vi "Finish Sequence.vi"(8 "error in":errorcluster, 11 "Sequence Executor in":refnum<class "Sequence Executor.lvclass">) -> (0 "error out":errorcluster, 3 "Sequence Executor out":refnum<class "Sequence Executor.lvclass">)   [LabVIEW 2026, in "Sequence Executor.lvclass"]
doc: "PRIVATE. Running F; verdict PASS iff every Step Result equals its step's expected_result; writes the CSV; applies safe setpoints to the rig; Status COMPLETE: verdict - file; refreshes displays."
uses:
  Sequence Executor.lvclass
  Sequence Executor.lvclass/Sequence Executor.ctl
  Rig Messages/Apply Setpoints Msg/Apply Setpoints Msg.lvclass/Apply Setpoints Msg.ctl
  <vilib>/ActorFramework/Message Enqueuer/Message Enqueuer.lvclass/Message Enqueuer.ctl
  <vilib>/ActorFramework/Message Enqueuer/Enqueue.vi
  Rig Messages/Apply Setpoints Msg/Apply Setpoints Msg.lvclass
  <vilib>/ActorFramework/Message Priority Queue/Priority Enqueue.vi
  <vilib>/ActorFramework/Message Enqueuer/Message Enqueuer.lvclass
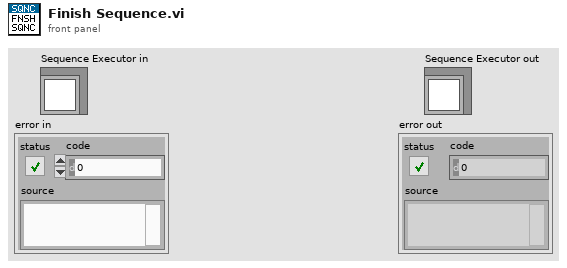
[diagram p1: front panel]
types:
  T1 = typedef "Step Result.ctl" = cluster{"step_no":i32, "step_name":string, "result":string, "reason":string, "measured":dbl, "target":dbl, "duration_ms":dbl}
  T2 = typedef "Sequence File.ctl" = cluster{"sequence_id":string, "description":string, "rig_config":string, "steps":T3[]}
  T3 = typedef "Step Config.ctl" = cluster{"step_no":i32, "step_name":string, "command_type":string, "setpoints":T4[], "conditions":T5[], "dwell_time_ms":i32, "timeout_ms":i32, "expected_result":string}
  T4 = typedef "Channel Value.ctl" = cluster{"channel":string, "value":dbl}
  T5 = typedef "Condition.ctl" = cluster{"channel":string, "target":dbl, "tolerance":dbl}
  T6 = typedef "Rig Config.ctl" = cluster{"rig_id":string, "description":string, "plugin_class":string, "channels":T7[]}
  T7 = typedef "Channel Definition.ctl" = cluster{"name":string, "unit":string, "min":dbl, "max":dbl}
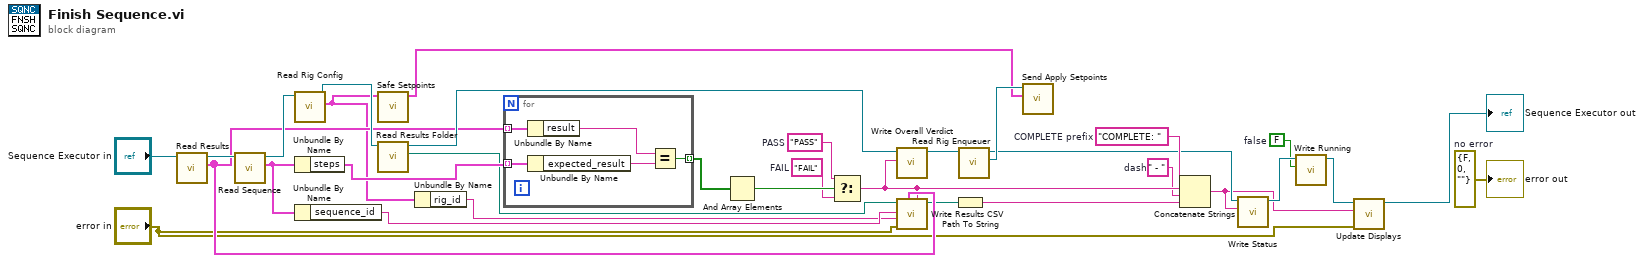
[diagram p0: block diagram]
diagram:
  w1 = FALSE  # false
  w10 = " - "  # dash
  w12 = "COMPLETE: "  # COMPLETE prefix
  w24 = "FAIL"  # FAIL
  w26 = "PASS"  # PASS
  w2 = errorcluster {"status"=FALSE, "code"=0, "source"=""}  # no error
  n1 = call "Read Results.vi"("Sequence Executor in"="Sequence Executor in") -> ("Results"=w18:T1[], "Sequence Executor out"=w31:refnum<class "Sequence Executor.lvclass">)  [unwired: 8 in, 1 out]
  n2 = call "Read Sequence.vi"("Sequence Executor in"=w31) -> ("Sequence File"=w22:T2, "Sequence Executor out"=w30:refnum<class "Sequence Executor.lvclass">)  [unwired: 8 in, 1 out]
  n3 = call "Read Rig Config.vi"("Sequence Executor in"=w30) -> ("Rig Config"=w17:T6, "Sequence Executor out"=w29:refnum<class "Sequence Executor.lvclass">)  [unwired: 8 in, 1 out]
  n4 = Unbundle By Name(w22) -> ("steps"=w28:T3[])
  n5 = Unbundle By Name(w22) -> ("sequence_id"=w20:string)
  n6 = call "Safe Setpoints.vi"("Rig Config"=w17) -> ("setpoints"=w14:cluster{"channel":string, "value":dbl}[])  [unwired: 10 in]
  n7 = call "Read Results Folder.vi"("Sequence Executor in"=w29) -> ("Results Folder"=w21:path, "Sequence Executor out"=w23:refnum<class "Sequence Executor.lvclass">)  [unwired: 8 in, 1 out]
  n8 = Unbundle By Name(w17) -> ("rig_id"=w19:string)
  n9 = for {
    tunnel: w18 -> [w37] mode=indexing
    tunnel: w28 -> [w36] mode=indexing
    tunnel: [w33] -> w27 mode=indexing
    n10 = Unbundle By Name(w37) -> ("result"=w35:string)
    n11 = Unbundle By Name(w36) -> ("expected_result"=w34:string)
    n12 = Equal?(x=w35, y=w34) -> (x = y?=w33:bool)
  }
  n13 = And Array Elements(Boolean array=w27) -> (logical AND=w25:bool)
  n14 = Select(t=w26, s=w25, f=w24) -> (s? t:f=w11:string)
  n15 = call "Write Overall Verdict.vi"("Overall Verdict"=w11, "Sequence Executor in"=w23) -> ("Sequence Executor out"=w16:refnum<class "Sequence Executor.lvclass">)  [unwired: 8 in, 1 out]
  n16 = call "Write Results CSV.vi"("overall verdict"=w11, "Step Results"=w18, "error in"="error in", "rig_id"=w19, "sequence_id"=w20, "results folder"=w21) -> ("file path"=w13:path)  [unwired: 4 in, 1 out]
  n17 = Path To String(path=w13) -> (string=w9:string)
  n18 = call "Read Rig Enqueuer.vi"("Sequence Executor in"=w16) -> ("Actor Framework:Message Enqueuer"=w15:refnum<class "Message Enqueuer.lvclass">, "Sequence Executor out"=w8:refnum<class "Sequence Executor.lvclass">)  [unwired: 8 in, 1 out]
  n19 = call "Send Apply Setpoints.vi"("setpoints"=w14, "Message Enqueuer"=w15) -> ()  [unwired: 8 in, 2 out]
  n20 = Concatenate Strings(w12, w11, w10, w9) -> (w5:string)
  n21 = call "Write Status.vi"("Status"=w5, "Sequence Executor in"=w8) -> ("Sequence Executor out"=w7:refnum<class "Sequence Executor.lvclass">)  [unwired: 8 in, 1 out]
  n22 = call "Write Running.vi"("Running"=w1, "Sequence Executor in"=w7) -> ("Sequence Executor out"=w6:refnum<class "Sequence Executor.lvclass">)  [unwired: 8 in, 1 out]
  n23 = call "Update Displays.vi"("error in"="error in", "Status"=w5, "Sequence Executor in"=w6) -> ("Sequence Executor out"=→"Sequence Executor out":refnum<class "Sequence Executor.lvclass">)  [unwired: 7 in, 1 out]
  "error out" <- w2
